vi "1_10_ScaleCar_HLV_enc.vi"() -> ()   [LabVIEW 2024]
uses:
  <vilib>/Instr/_visa.llb/VISA Set IO Buffer Mask.ctl
  <vilib>/Instr/_visa.llb/VISA Flush IO Buffer Mask.ctl
  <vilib>/Instr/_visa.llb/VISA Configure Serial Port (Instr).vi
panel:
  out "PCU_ENC":i32
  out "ARD_EStop":u8
  in  "HLV_EStop":bool
  out "PCU_MODE":u8
  out "PCU_GEAR":u8
  in  "HLV_GEAR":u8(slide)=1 scale=0.0..2.0
  out "string":string
  out "TX Data Cnt (byte)":u32
  out "RX Data Cnt (byte)":u32
  in  "HLV_SPEED":i16(slide) scale=0.0..1000.0
  out "하위제어기 통신 패킷":string
  in  "HLV_AorM":bool
  out "PCU_ALIVE":u8
  out "PCU_STEER":i16
  out "PCU_SPEED (mps)":dbl
  in  "Serial Name":refnum<visa-resource-name>="COM1"
  in  "stop":bool
  # "1/10_RACING TEST PROGRAM"
  # "20210814_by. KBS"
  # "Control"
  # "Feedback"
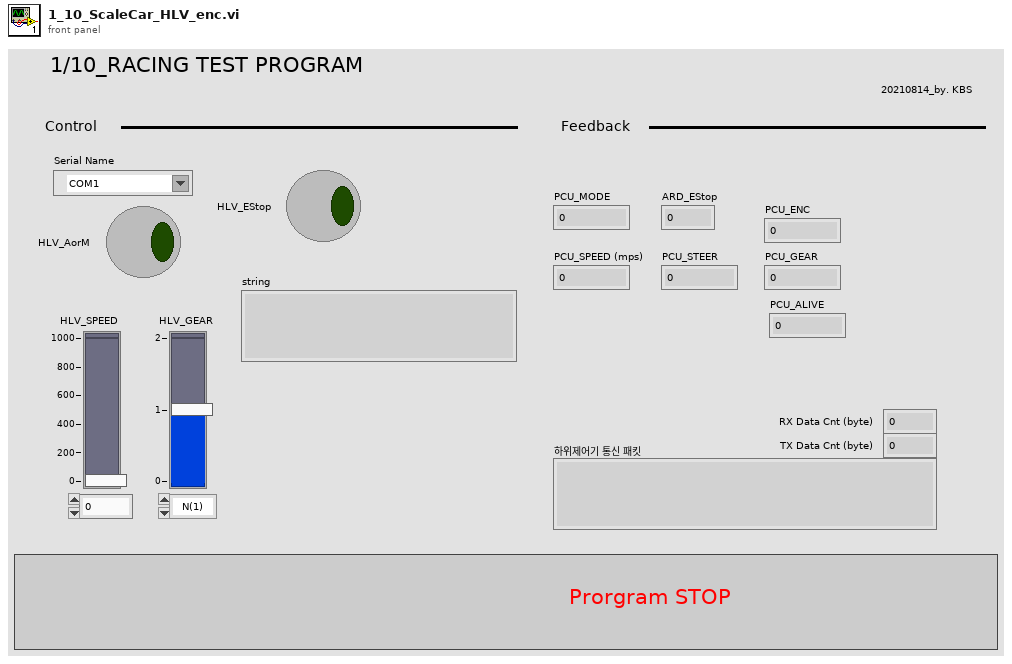
[diagram p1: front panel]
types:
  T1 = typedef "VISA Flush IO Buffer Mask.ctl" = u16
  T2 = typedef "VISA Set IO Buffer Mask.ctl" = u16
  T3 = cluster{"HLV_M/A_Status":u8, "HLV_EStop":u8, "HLV_Gear":u8, "HLV_Speed":i16, "HLV_Steer":i16, "HLV_Alive":u8}
  T4 = cluster{"ARD_M/A_Status":u8, "ARD_EStop":u8, "ARD_Gear":u8, "ARD_Speed":i16, "ARD_Steer":i16, "ARD_ENC":i32, "ARD_Alive":u8}
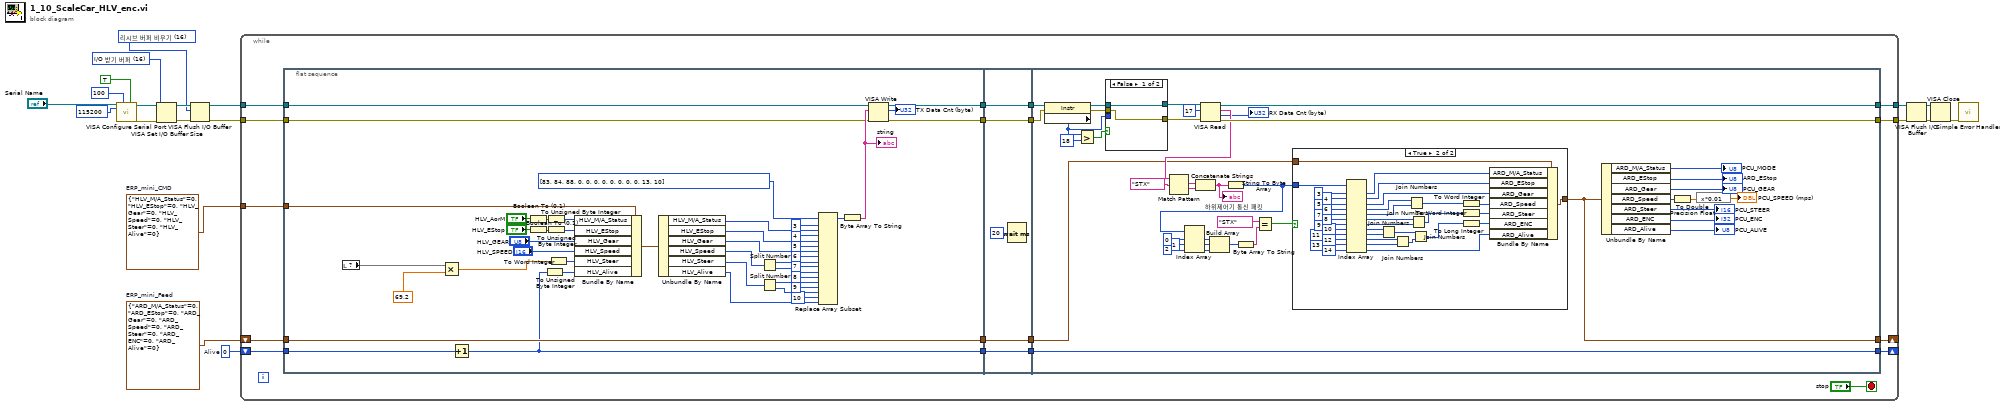
[diagram p0: block diagram]
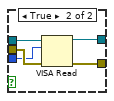
[diagram p2: hidden frame]
diagram:
  w1 = u8 0  # Alive
  w4 = T1 16 items=["리시브 버퍼 비우기"=16, "전달 버퍼 디바이스에 쓰기"=32, "리시브 버퍼 비우기(I/O 없음)"=64, "전달 버퍼 비우기"=128] ("Mask")
  w7 = T2 16 items=["I/O 받기 버퍼"=16, "I/O 전달 버퍼"=32, "I/O 받기와 전달 버퍼"=48] ("Mask")
  w13 = T3 {"HLV_M/A_Status"=0, "HLV_EStop"=0, "HLV_Gear"=0, "HLV_Speed"=0, "HLV_Steer"=0, "HLV_Alive"=0}  # ERP_mini_CMD
  w14 = T4 {"ARD_M/A_Status"=0, "ARD_EStop"=0, "ARD_Gear"=0, "ARD_Speed"=0, "ARD_Steer"=0, "ARD_ENC"=0, "ARD_Alive"=0}  # ERP_mini_Feed
  n1 = call-poly "VISA Configure Serial Port"("VISA resource name"="Serial Name", "timeout (10sec)"=u32 100, "Enable Termination\nChar (T)"=TRUE ("Enable Termination\nChar (T)"), "baud rate (9600)"=u32 115200) -> ("VISA resource name out"=w9:refnum<visa-resource-name>, "error out"=w8:errorcluster)  [unwired: 10 in]
  n2 = VISA Set I/O Buffer Size(VISA resource name=w9, mask (16)=w7, error in (no error)=w8) -> (VISA resource name out=w6:refnum<visa-resource-name>, error out=w5:errorcluster)  [unwired: 1 in]
  n3 = VISA Flush I/O Buffer(VISA resource name=w6, mask (16)=w4, error in (no error)=w5) -> (VISA resource name out=w18:refnum<visa-resource-name>, error out=w2:errorcluster)
  n4 = while {
    tunnel: w18 -> [w37]
    tunnel: w2 -> [w36]
    tunnel: [w31] -> w17
    tunnel: [w30] -> w16
    shift-right: [w26] -> _
    shift-left: w14 -> [w28]
    tunnel: w13 -> [w25]
    shift-right: [w21] -> _
    shift-left: w1 -> [w24]
    stop <- "stop" stop-if-true
    n5 = flat-sequence {
      tunnel: [w68] -> w34
      tunnel: [w67] -> w32
      tunnel: w37 -> [w70]
      tunnel: w36 -> [w69]
      tunnel: [w65] -> w29
      tunnel: w28 -> [w65]
      tunnel: w25 -> [w64]
      tunnel: w24 -> [w61]
      tunnel: [w60] -> w22
      tunnel: [w87] -> w35
      tunnel: w34 -> [w87]
      tunnel: [w86] -> w33
      tunnel: w32 -> [w86]
      tunnel: w29 -> [w85]
      tunnel: [w85] -> w27
      tunnel: [w84] -> w23
      tunnel: w22 -> [w84]
      tunnel: w35 -> [w106]
      tunnel: w33 -> [w105]
      tunnel: [w128] -> w31
      tunnel: [w127] -> w30
      tunnel: w27 -> [w108]
      tunnel: [w107] -> w26
      tunnel: [w97] -> w21
      tunnel: w23 -> [w97]
      frame #0 {
        n6 = local read item#-1() -> (w41)
        n7 = Multiply(x=w41, y=69.2) -> (x*y=w39:dbl)
        n8 = Increment(x=w61) -> (x+1=w60:u8)
        n9 = Boolean To (0,1)(Boolean="HLV_AorM") -> (0, 1=w62:i16)
        n10 = Boolean To (0,1)(Boolean="HLV_EStop") -> (0, 1=w53:i16)
        n11 = To Unsigned Byte Integer(number=w60) -> (unsigned 8bit integer=w76:u8)
        n12 = To Unsigned Byte Integer(number=w62) -> (unsigned 8bit integer=w54:u8)
        n13 = To Unsigned Byte Integer(number=w53) -> (unsigned 8bit integer=w51:u8)
        n14 = To Word Integer(number=w39) -> (16bit integer=w63:i16)
        n15 = Bundle By Name(cluster=w64, "HLV_M/A_Status"=w54, "HLV_EStop"=w51, "HLV_Gear"="HLV_GEAR", "HLV_Speed"="HLV_SPEED", "HLV_Steer"=w63, "HLV_Alive"=w76) -> (w71:T3)
        n16 = Unbundle By Name(w71) -> ("HLV_M/A_Status"=w50:u8, "HLV_EStop"=w49:u8, "HLV_Gear"=w48:u8, "HLV_Speed"=w56:i16, "HLV_Steer"=w55:i16, "HLV_Alive"=w42:u8)
        n17 = Split Number(x=w56) -> (hi(x)=w47:u8, lo(x)=w46:u8)
        n18 = Split Number(x=w55) -> (hi(x)=w45:u8, lo(x)=w44:u8)
        n19 = Replace Array Subset(array=u8[] [83, 84, 88, 0, 0, 0, 0, 0, 0, 0, 0, 13, 10] ("unsigned byte array"), new element #1=w50, index #1=3, new element #2=w49, index #2=4, new element #3=w48, index #3=5, new element #4=w47, index #4=6, new element #5=w46, index #5=7, new element #6=w45, index #6=8, new element #7=w44, index #7=9, new element #8=w42, index #8=10) -> (w80:u8[])
        n20 = Byte Array To String(unsigned byte array=w80) -> (string=w81:string)
        "string" <- w81
        n21 = VISA Write(VISA resource name=w70, write buffer=w81, error in (no error)=w69) -> (VISA resource name out=w68:refnum<visa-resource-name>, return count=→"TX Data Cnt (byte)":u32, error out=w67:errorcluster)
      }
      frame #1 {
        n22 = Wait (ms)(milliseconds to wait=u32 20 ("대기 시간 (ms)")) -> ()  [unwired: 1 out]
      }
      frame #2 {
        n23 = property class="Instr"(reference=w106, error in=w105) -> (reference out=w104:refnum<visa-resource-name>, error out=w103:errorcluster, "Serial Settings:Number of Bytes at Serial Port"=w98:u32)
        n24 = Greater?(x=w98, y=u32 18) -> (0:w100:bool)
        n25 = case shown="False" w100 {
          tunnel: w104 -> [w130 w135]
          tunnel: w103 -> [w129 w134]
          tunnel: [w130 w133] -> w102
          tunnel: [w129 w132] -> w101
          tunnel: w98 -> [_ w131]
          frame False {
          }
          frame True {
            n26 = VISA Read(VISA resource name=w135, byte count=w131, error in (no error)=w134) -> (VISA resource name out=w133:refnum<visa-resource-name>, error out=w132:errorcluster)  [unwired: 2 out]
          }
        }
        n27 = VISA Read(VISA resource name=w102, byte count=u32 17, error in (no error)=w101) -> (VISA resource name out=w128:refnum<visa-resource-name>, read buffer=w126:string, return count=→"RX Data Cnt (byte)":u32, error out=w127:errorcluster)
        n28 = Match Pattern(string=w126, regular expression="STX") -> (match substring=w123:string, after substring=w124:string)  [unwired: 1 in, 2 out]
        n29 = Concatenate Strings(w123, w124) -> (w122:string)
        "하위제어기 통신 패킷" <- w122
        n30 = String To Byte Array(string=w122) -> (unsigned byte array=w110:u8[])
        n31 = Index Array(array=w110, index #1=0, index #2=1, index #3=2) -> (element #1=w116:u8, element #2=w115:u8, element #3=w114:u8)
        n32 = Build Array(w116, w115, w114) -> (w113:u8[])
        n33 = Byte Array To String(unsigned byte array=w113) -> (string=w111:string)
        n34 = Equal?(x="STX", y=w111) -> (x = y?=w109:bool)
        n35 = case shown="True" w109 {
          tunnel: w110 -> [_ w171]
          tunnel: [w136 w170] -> w107
          tunnel: w108 -> [w136 w169]
          frame False {
          }
          frame True {
            n36 = Index Array(array=w171, index #1=3, index #2=4, index #3=5, index #4=6, index #5=7, index #6=8, index #7=9, index #8=10, index #9=11, index #10=12, index #11=13, index #12=14) -> (element #1=w158:u8, element #2=w157:u8, element #3=w156:u8, element #4=w155:u8, element #5=w154:u8, element #6=w152:u8, element #7=w151:u8, element #8=w143:u8, element #9=w142:u8, element #10=w141:u8, element #11=w140:u8, element #12=w145:u8)
            n37 = Join Numbers(hi=w143, lo=w142) -> ((hi.lo)=w139:u16)
            n38 = Join Numbers(hi=w141, lo=w140) -> ((hi.lo)=w138:u16)
            n39 = Join Numbers(hi=w155, lo=w154) -> ((hi.lo)=w153:u16)
            n40 = Join Numbers(hi=w152, lo=w151) -> ((hi.lo)=w150:u16)
            n41 = Join Numbers(hi=w139, lo=w138) -> ((hi.lo)=w137:u32)
            n42 = To Word Integer(number=w153) -> (16bit integer=w162:i16)
            n43 = To Word Integer(number=w150) -> (16bit integer=w161:i16)
            n44 = To Long Integer(number=w137) -> (32bit integer=w144:i32)
            n45 = Bundle By Name(cluster=w169, "ARD_M/A_Status"=w158, "ARD_EStop"=w157, "ARD_Gear"=w156, "ARD_Speed"=w162, "ARD_Steer"=w161, "ARD_ENC"=w144, "ARD_Alive"=w145) -> (w170:T4)
          }
        }
        n46 = Unbundle By Name(w107) -> ("ARD_M/A_Status"=→"PCU_MODE":u8, "ARD_EStop"=→"ARD_EStop":u8, "ARD_Gear"=→"PCU_GEAR":u8, "ARD_Speed"=w94:i16, "ARD_Steer"=→"PCU_STEER":i16, "ARD_ENC"=→"PCU_ENC":i32, "ARD_Alive"=→"PCU_ALIVE":u8)
        n47 = To Double Precision Float(number=w94) -> (double precision float=w95:dbl)
        n48 = expression code="x*0.01"(w95) -> (→"PCU_SPEED (mps)":dbl)
      }
    }
  }
  n49 = VISA Flush I/O Buffer(VISA resource name=w17, error in (no error)=w16) -> (VISA resource name out=w19:refnum<visa-resource-name>, error out=w20:errorcluster)  [unwired: 1 in]
  n50 = VISA Close(VISA resource name=w19, error in (no error)=w20) -> (error out=w15:errorcluster)
  n51 = call <vilib>:"Simple Error Handler.vi"("error in (no error)"=w15) -> ()  [unwired: 4 in, 5 out]
